vi "Folder Drag_and_Drop.vi"(10 "リング":u16(ring)) -> (3 "Folder_Name":path)   [LabVIEW 2018]
panel:
  in  "パス":path
  in  "Insert":bool
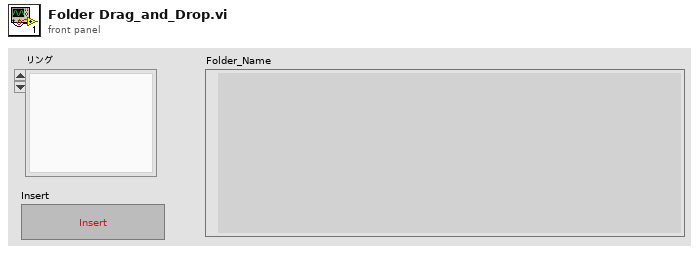
[diagram p1: front panel]
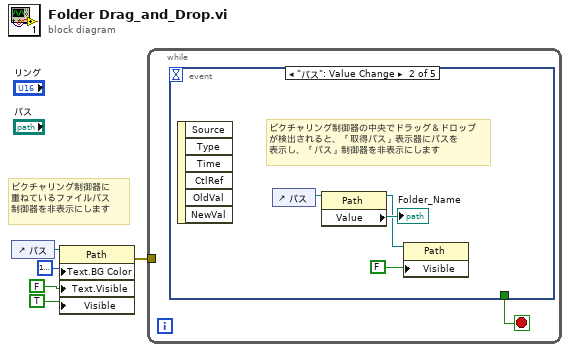
[diagram p0: block diagram]
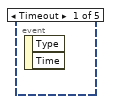
[diagram p2: hidden frame]
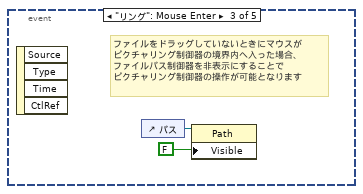
[diagram p3: hidden frame]
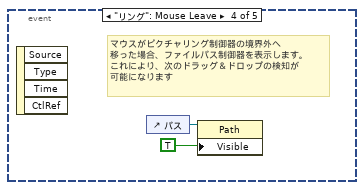
[diagram p4: hidden frame]
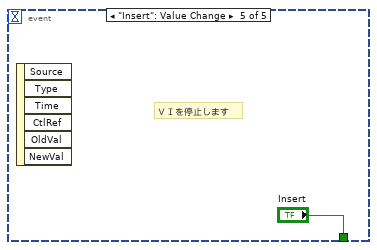
[diagram p5: hidden frame]
diagram:
  # "ピクチャリング制御器に\n重ねているファイルパス\n制御器を非表示にします"
  n1 = control-ref of="パス"() -> (w2:refnum<vi>)
  n2 = property class="Path"(reference=w2, "Text.BG Color"=u32 16777216, "Text.Visible"=FALSE ("Path Text.Visible"), "Visible"=TRUE) -> (error out=w1:errorcluster)  [unwired: 1 in, 1 out]
  n3 = while {
    tunnel: w1 -> [_]
    stop <- w6 stop-if-true
    n4 = event shown="[1] \"パス\": Value Change" {
      selector: _ -> [_ _ _ _ _]
      dyn-events: _ -> [_ _ _ _ _]
      timeout: _ -> [_ _ _ _ _]
      tunnel: [_ _ _ _ "Insert"] -> w6
      event Timeout {
        n5 = event-data() -> ()  [unwired: 1 in, 2 out]
      }
      event "パス": Value Change {
        # "ピクチャリング制御器の中央でドラッグ＆ドロップ\nが検出されると、「取得パス」表示器にパスを\n表示し、「パス」制御器を非表示にします"
        n6 = event-data() -> ()  [unwired: 1 in, 6 out]
        n7 = control-ref of="パス"() -> (w9:refnum<vi>)
        n8 = property class="Path"(reference=w9) -> (reference out=w7:refnum<vi>, "Value"=→"Folder_Name":path)  [unwired: 1 in, 1 out]
        n9 = property class="Path"(reference=w7, "Visible"=FALSE) -> ()  [unwired: 1 in, 2 out]
      }
      event "リング": Mouse Enter {
        # "ファイルをドラッグしていないときにマウスが\nピクチャリング制御器の境界内へ入った場合、\nファイルパス制御器を非表示にすることで\nピクチャリング制御器の操作が可能となります"
        n10 = event-data() -> ()  [unwired: 1 in, 4 out]
        n11 = control-ref of="パス"() -> (w11:refnum<vi>)
        n12 = property class="Path"(reference=w11, "Visible"=FALSE) -> ()  [unwired: 1 in, 2 out]
      }
      event "リング": Mouse Leave {
        # "マウスがピクチャリング制御器の境界外へ\n移った場合、ファイルパス制御器を表示します。\nこれにより、次のドラッグ＆ドロップの検知が\n可能になります"
        n13 = event-data() -> ()  [unwired: 1 in, 4 out]
        n14 = control-ref of="パス"() -> (w14:refnum<vi>)
        n15 = property class="Path"(reference=w14, "Visible"=TRUE) -> ()  [unwired: 1 in, 2 out]
      }
      event "Insert": Value Change {
        # "ＶＩを停止します"
        n16 = event-data() -> ()  [unwired: 1 in, 6 out]
      }
    }
  }
